vi "Native_SetLoopTunnelIndexMode.vi"() -> ()   [LabVIEW 2024]
panel:
  out "error out":errorcluster caption="错误输出"
  in  "index_mode":u32
  in  "tunnel_id":u32
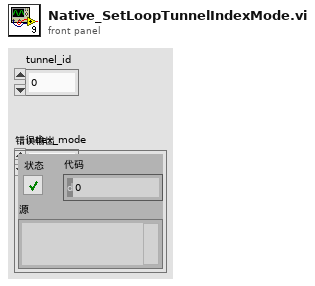
[diagram p1: front panel]
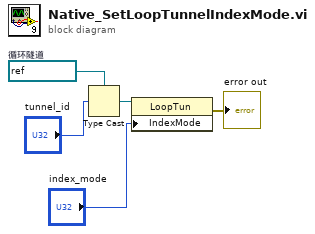
[diagram p0: block diagram]
diagram:
  w4 = refnum<vi> refnum  # 循环隧道
  n1 = Type Cast ("强制类型转换")(type=w4, x="tunnel_id") -> (*(type *) &x=w3:refnum<vi>)
  n2 = property on="属性节点" class="LoopTun"(reference=w3, "IndexMode"="index_mode") -> (error out=→"error out":errorcluster)  [unwired: 1 in, 1 out]
